vi "Test_REST_Call.vi"() -> ()   [LabVIEW 2021]
uses:
  common/CANsub_Common.lvlib
  <vilib>/httpClient/LabVIEWHTTPClient.lvlib
  common/Typedefs/HTTP_Method.ctl
panel:
  out "response":string
  out "status":i32
  out "error out":errorcluster
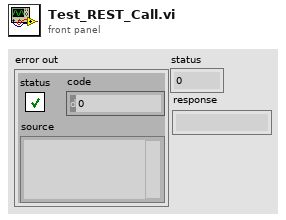
[diagram p1: front panel]
types:
  T1 = typedef "CANsub_Common.lvlib/HTTP_Method.ctl" = enum16{"GET", "PUT", "POST", "DELETE"}
  T2 = typedef "LabVIEWHTTPClient.lvlib/ClientHandle.ctl" = refnum<k1>
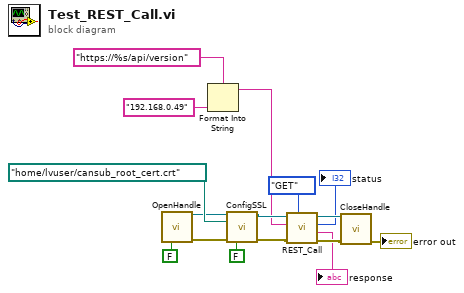
[diagram p0: block diagram]
diagram:
  n1 = call <vilib>:"OpenHandle.vi"("verify server(true)"=FALSE) -> ("client handle out"=w2:T2, "error out"=w16:errorcluster)  [unwired: 13 in]
  n2 = Format Into String(format string="https://%s/api/version", "192.168.0.49" ("url")) -> (resulting string=w3:string)  [unwired: 2 in, 1 out]
  n3 = call <vilib>:"ConfigSSL.vi"("client handle"=w2, "CA certificate file"=path "/home/lvuser/cansub_root_cert.crt" ("client certificate file"), "error in (no error)"=w16, "verify server (true)"=FALSE) -> ("client handle out"=w10:T2, "error out"=w15:errorcluster)  [unwired: 10 in]
  n4 = call "REST_Call.vi"("method"=HTTP_Method."GET", "error in (no error)"=w15, "url"=w3, "client handle"=w10) -> ("error out"=w14:errorcluster, "response"=→"response":string, "status"=→"status":i32, "client handle out"=w8:T2)  [unwired: 4 in]
  n5 = call <vilib>:"CloseHandle.vi"("client handle"=w8, "error in (no error)"=w14) -> ("error out"=→"error out":errorcluster)  [unwired: 13 in]
